vi "Label of Cluster in Type Definition Template--constant.vi"() -> (3 "Label of Cluster in Type Definition Template":string)   [LabVIEW 2026]
doc: "Label of cluster in template."
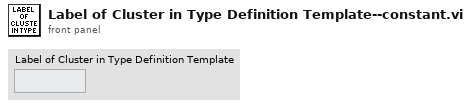
[diagram p1: front panel]
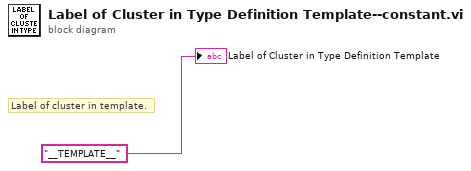
[diagram p0: block diagram]
diagram:
  # "Label of cluster in template."
  "Label of Cluster in Type Definition Template" <- "__TEMPLATE__" ("Label of Cluster in Type Definition Template")
